vi "Set Cell Text.vi"(7 "Sheet Name":string="table2", 8 "error in (no error)":errorcluster, 9 "position":cluster{"Row":i32, "Column":i32}={"Row"=1, "Column"=1}, 10 "text":string, 11 "report in":refnum<class "ooCalc.lvclass">) -> (0 "error out":errorcluster, 3 "report out":refnum<class "ooCalc.lvclass">)   [LabVIEW 2009, in "ooCalc.lvclass"]
doc: "Appends text to the selected report."
uses:
  ooCalc.lvclass
  C:/Projets/LAVAG/OpenOfficeRGT/AODL/DLLs/AODL.dll
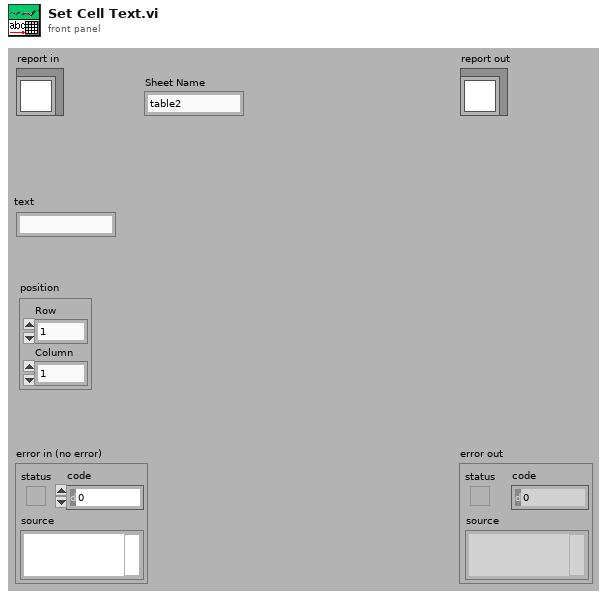
[diagram p1: front panel]
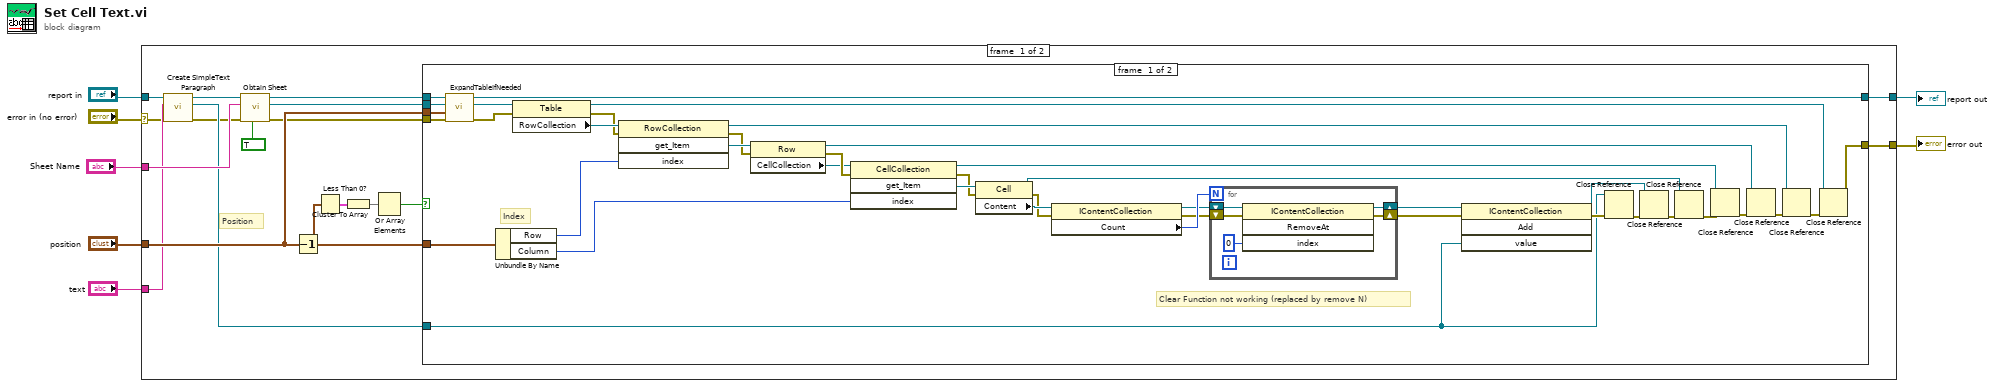
[diagram p0: block diagram]
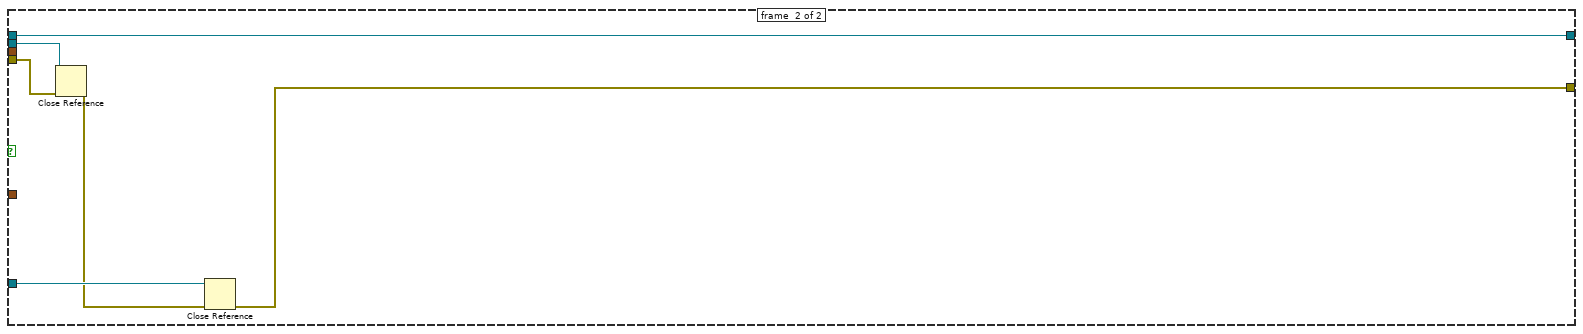
[diagram p2: hidden frame]
diagram:
  n1 = case shown="No Error" "error in (no error)" {
    selector: "error in (no error)" -> [w14 w77]
    tunnel: [w20 w77] -> w5
    tunnel: [w9 w76] -> w6
    tunnel: "report in" -> [w18 w76]
    tunnel: "text" -> [w19 _]
    tunnel: "Sheet Name" -> [w25 _]
    tunnel: "position" -> [w22 _]
    frame #0 {
      # "Position"
      n2 = call-dynamic "Create SimpleText Paragraph.vi"("error in (no error)"=w14, "simpleText"=w19, "ooCalc in"=w18) -> ("error out"=w15:errorcluster, "SimpleTextParagraph"=w17:refnum<k24>, "ooCalc out"=w16:refnum<class "ooCalc.lvclass">)  [unwired: 6 in]
      n3 = call-dynamic "Obtain Sheet.vi"("Create if non-existant? (T)"=TRUE, "error in (no error)"=w15, "Sheet Name"=w25, "ooCalc in"=w16) -> ("error out"=w21:errorcluster, "Sheet"=w23:refnum<k24>, "ooCalc out"=w10:refnum<class "ooCalc.lvclass">)  [unwired: 5 in]
      n4 = Decrement(x=w22) -> (x-1=w13:cluster{"Row":i32, "Column":i32})
      n5 = Less Than 0?(x=w13) -> (x < 0?=w12:cluster{"Row":bool, "Column":bool})
      n6 = Cluster To Array(cluster=w12) -> (array=w11:bool[])
      n7 = Or Array Elements(Boolean array=w11) -> (logical OR=w8:bool)
      n8 = case shown="False" w8 {
        tunnel: w23 -> [w64 w73]
        tunnel: w22 -> [w58 _]
        tunnel: w21 -> [w51 w72]
        tunnel: [w39 w70] -> w20
        tunnel: w17 -> [w29 w74]
        tunnel: w13 -> [w27 _]
        tunnel: w10 -> [w26 w75]
        tunnel: [w26 w75] -> w9
        frame #0 {
          # "Clear Function not working (replaced by remove N)"
          # "Index"
          n9 = call "ExpandTableIfNeeded.vi"("error in"=w51, "Table Size"=w58, "Table in"=w64) -> ("error out"=w54:errorcluster, "Table out"=w61:refnum<k24>)  [unwired: 7 in]
          n10 = Unbundle By Name(w27) -> ("Row"=w56:i32, "Column"=w57:i32)
          n11 = property on="Property Node" class="Table"(reference=w61, error in=w54) -> (reference out=w40:refnum<k24>, error out=w59:errorcluster, "RowCollection"=w60:refnum<k24>)
          n12 = invoke class="RowCollection" method="get_Item"(reference=w60, error in=w59, "index"=w56) -> (reference out=w42:refnum<k24>, error out=w52:errorcluster, "get_Item"=w55:refnum<k24>)  [unwired: 1 in, 1 out]
          n13 = property on="Property Node" class="Row"(reference=w55, error in=w52) -> (reference out=w43:refnum<k24>, error out=w53:errorcluster, "CellCollection"=w50:refnum<k24>)
          n14 = invoke class="CellCollection" method="get_Item"(reference=w50, error in=w53, "index"=w57) -> (reference out=w44:refnum<k24>, error out=w62:errorcluster, "get_Item"=w63:refnum<k24>)  [unwired: 1 in, 1 out]
          n15 = property on="Property Node" class="Cell"(reference=w63, error in=w62) -> (reference out=w31:refnum<k24>, error out=w34:errorcluster, "Content"=w37:refnum<k24>)
          n16 = property on="Property Node" class="IContentCollection"(reference=w37, error in=w34) -> (reference out=w36:refnum<k24>, error out=w35:errorcluster, "Count"=w38:i32)
          n17 = for {
            N: w38 -> [_]
            shift-right: [w69] -> w33
            shift-left: w36 -> [w66]
            shift-right: [w68] -> w32
            shift-left: w35 -> [w67]
            n18 = invoke class="IContentCollection" method="RemoveAt"(reference=w66, error in=w67, "index"=0) -> (reference out=w69:refnum<k24>, error out=w68:errorcluster)  [unwired: 1 in, 2 out]
          }
          n19 = invoke class="IContentCollection" method="Add"(reference=w33, error in=w32, "value"=w29) -> (reference out=w47:refnum<k24>, error out=w30:errorcluster)  [unwired: 1 in, 2 out]
          n20 = Close Reference(reference=w29, error in (no error)=w30) -> (error out=w49:errorcluster)
          n21 = Close Reference(reference=w47, error in (no error)=w49) -> (error out=w48:errorcluster)
          n22 = Close Reference(reference=w31, error in (no error)=w48) -> (error out=w28:errorcluster)
          n23 = Close Reference(reference=w44, error in (no error)=w28) -> (error out=w46:errorcluster)
          n24 = Close Reference(reference=w43, error in (no error)=w46) -> (error out=w45:errorcluster)
          n25 = Close Reference(reference=w42, error in (no error)=w45) -> (error out=w41:errorcluster)
          n26 = Close Reference(reference=w40, error in (no error)=w41) -> (error out=w39:errorcluster)
        }
        frame #1 {
          n27 = Close Reference(reference=w73, error in (no error)=w72) -> (error out=w71:errorcluster)
          n28 = Close Reference(reference=w74, error in (no error)=w71) -> (error out=w70:errorcluster)
        }
      }
    }
    frame #1 {
    }
  }
  "error out" <- w5
  "report out" <- w6
